vi "Remove Invalid DMAs.vi"(8 "error in (no error)":errorcluster, 9 "invalid DMA channels":T1[](array[typedef]) {"Data Type" format="%.0x"}, 10 "section name":string, 11 "item ref in":T3 format="%.0x") -> (0 "error out":errorcluster, 3 "item ref out":T3 format="%.0x")   [LabVIEW 2020, in "FPGA Addon System Explorer.lvlib"]
uses:
  FPGA Addon System Explorer.lvlib
  <vilib>/NI VeriStand/Custom Device API/Custom Device Item Ref.ctl
  Addon Shared/Types/DMA Information.ctl
  Addon Shared/Types/FPGA Addon Data Type.ctl
  <vilib>/NI VeriStand/Custom Device Tools/Custom Device Utility Library/NI VeriStand - Search for Item by Name.vi
  <vilib>/NI VeriStand/Custom Device Tools/Custom Device Utility Library/Custom Device Utility Library.lvlib
  <vilib>/NI VeriStand/Custom Device API/Custom Device API.lvlib
  Addon Shared/FPGA Addon Shared.lvlib
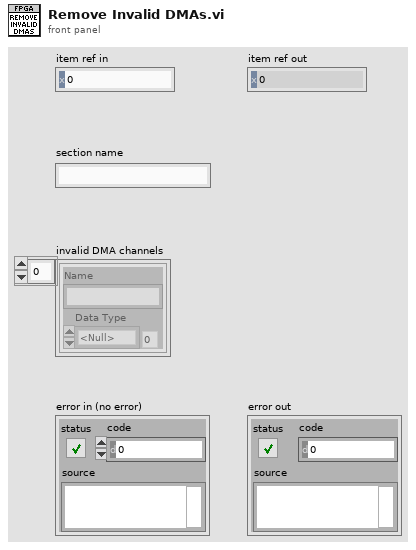
[diagram p1: front panel]
types:
  T1 = typedef "FPGA Addon Shared.lvlib/DMA Information.ctl" = cluster{"Name":string, "Data Type":T2}
  T2 = typedef "FPGA Addon Shared.lvlib/FPGA Addon Data Type.ctl" = enum8{"<Null>", "I8", "I16", "I32", "I64", "U8", "U16", "U32", "U64", "SGL", "Boolean", "Analog PWM In Settings", "Analog PWM In", "Digital PWM In Settings", "Digital PWM In", "Digital PWM Out", "Sine Out", "FXP", "FXP+/-24.5", "FXP+/-16.5", "FXP+/-32.8", "FXP+/-64.32", "FXP+/-16.7", "FXP+/-20.5", "FXP+/-27.5", "FXP+/-32.16", "FXP+16.3", "FXP+18.3", "Digital Static In", "Digital Static Out", "Digital Static In Settings", "Digital WSS Out", "Quad Encoder Settings", "Quad Encoder In", "Group"}
  T3 = typedef "Custom Device API.lvlib/Custom Device Item Ref.ctl" = u64
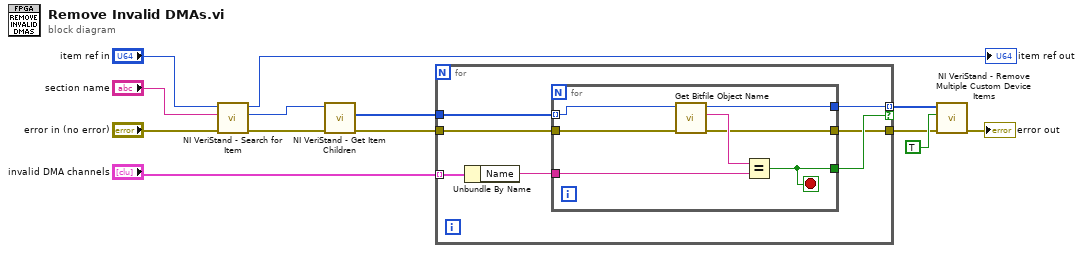
[diagram p0: block diagram]
diagram:
  n1 = call-poly <vilib>:"NI VeriStand - Search for Item.vi"("error in"="error in (no error)", "Item Name"="section name", "Section Ref in"="item ref in") -> ("error out"=w4:errorcluster, "Item Ref"=w3:T3, "Section Ref out"=→"item ref out":T3)  [unwired: 5 in, 1 out]
  n2 = call <vilib>:"NI VeriStand - Get Item Children.vi"("error in (no error)"=w4, "Item Ref in"=w3) -> ("error out"=w2:errorcluster, "Child Refs"=w1:T3[])  [unwired: 6 in, 2 out]
  n3 = for {
    tunnel: "invalid DMA channels" -> [w20] mode=indexing
    tunnel: [w19] -> w8 mode=indexing if=w17
    tunnel: w2 -> [w16]
    tunnel: w1 -> [w15]
    tunnel: [w14] -> w5
    n4 = Unbundle By Name(w20) -> ("Name"=w18:string)
    n5 = for {
      tunnel: [w27] -> w19
      tunnel: w18 -> [w26]
      tunnel: [w21] -> w17
      tunnel: w16 -> [w24]
      tunnel: w15 -> [w23] mode=indexing
      tunnel: [w22] -> w14
      stop <- w21 stop-if-true
      n6 = call "Get Bitfile Object Name.vi"("error in (no error)"=w24, "Item Ref in"=w23) -> ("error out"=w22:errorcluster, "Value"=w25:string, "Item Ref out"=w27:T3)  [unwired: 7 in]
      n7 = Equal?(x=w25, y=w26) -> (x = y?=w21:bool)
    }
  }
  n8 = call <vilib>:"NI VeriStand - Remove Multiple Custom Device Items.vi"("error in (no error)"=w5, "Force Delete (F)"=TRUE, "Item Refs in"=w8) -> ("error out"=→"error out":errorcluster)  [unwired: 7 in, 1 out]
